vi "SpeedTokenizer.vi"(8 "error in (no error)":errorcluster, 11 "Command String":string) -> (0 "error out":errorcluster, 3 "Tokens":string[](array[string]))   [LabVIEW 2019, in "PathTokenizer.lvclass"]
uses:
  PathTokenizer.lvclass
  <vilib>/Utility/error.llb/whitespace.ctl
  <vilib>/regexp/Match Regular Expression.xnode
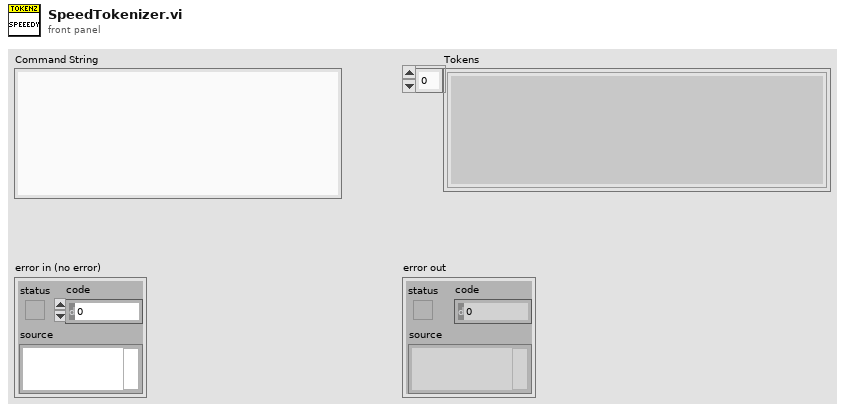
[diagram p1: front panel]
types:
  T1 = typedef "whitespace.ctl" = u16
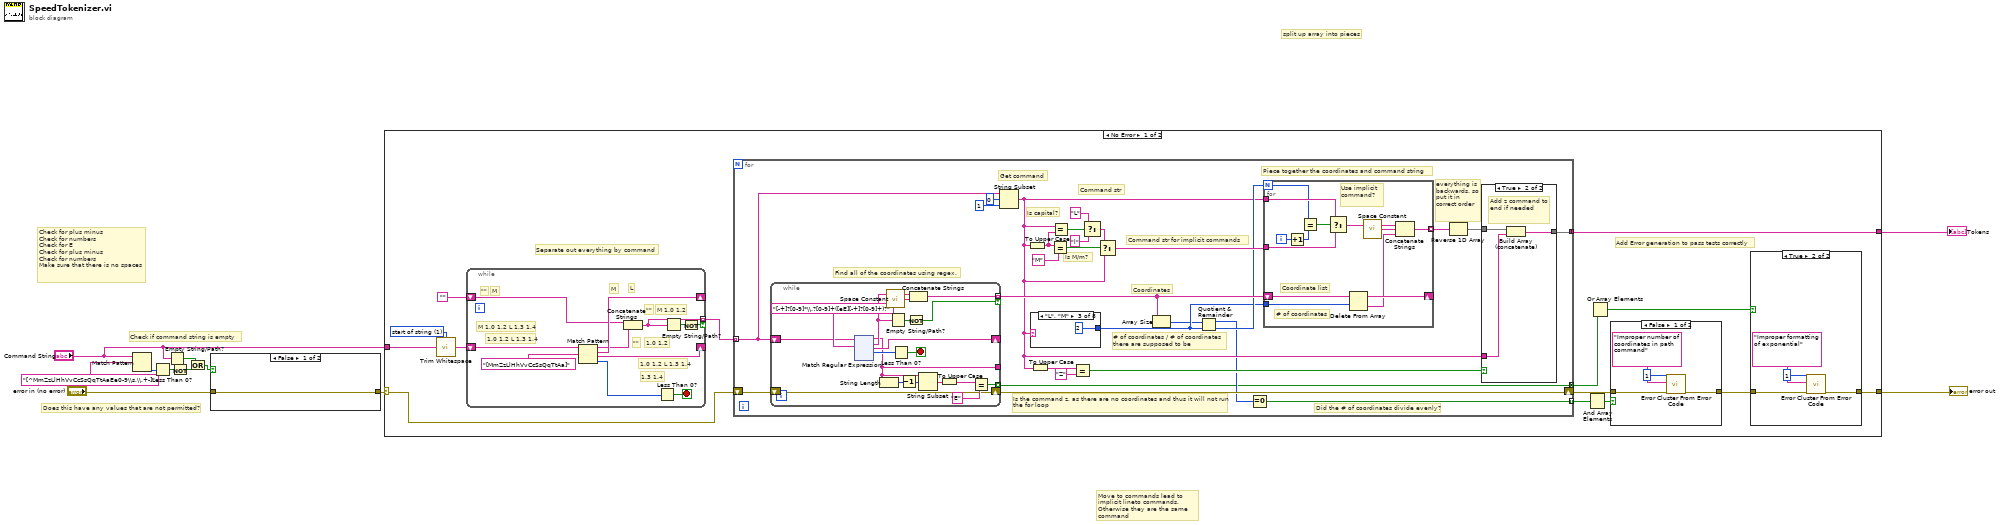
[diagram p0: block diagram]
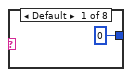
[diagram p5: hidden frame]
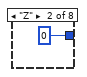
[diagram p6: hidden frame]
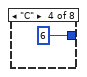
[diagram p7: hidden frame]
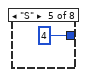
[diagram p8: hidden frame]
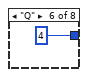
[diagram p9: hidden frame]
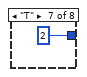
[diagram p10: hidden frame]
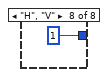
[diagram p11: hidden frame]
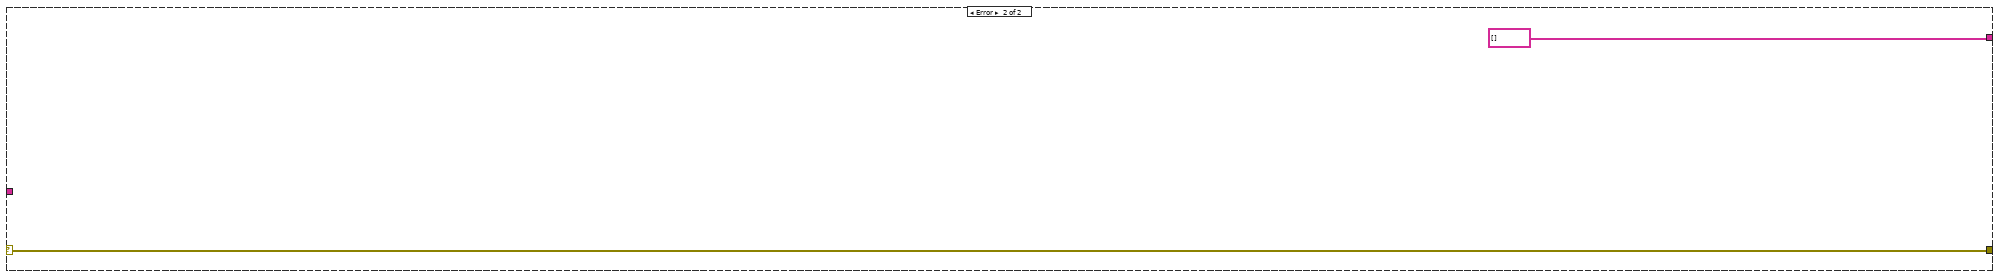
[diagram p12: hidden frame]
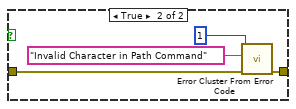
[diagram p13: hidden frame]
diagram:
  # "Check if command string is empty"
  # "Does this have any values that are not permitted?"
  # "Move to commands lead to implicit lineto commands. Otherwise they are the same command"
  # "split up array into pieces"
  # "Check for plus minus\nCheck for numbers\nCheck for E\nCheck for plus minus\nCheck for numbers\nMake sure that there is no spaces"
  n1 = Match Pattern(string="Command String", regular expression="[^MmZzLlHhVvCcSsQqTtAaEe0-9\\s,\\.+-]") -> (offset past match=w9:i32)  [unwired: 1 in, 3 out]
  n2 = Less Than 0?(x=w9) -> (x < 0?=w5:bool)
  n3 = Empty String/Path?(string/path="Command String") -> (empty?=w2:bool)
  n4 = Not(x=w5) -> (.not. x?=w4:bool)
  n5 = Or(x=w2, y=w4) -> (x .or. y?=w3:bool)
  n6 = case shown="False" w3 {
    tunnel: "error in (no error)" -> [w12 w14]
    tunnel: [w12 w13] -> w6
    frame False {
    }
    frame True {
      n7 = call <vilib>:"Error Cluster From Error Code.vi"("error in (no error)"=w14, "error message (\"\")"="Invalid Character in Path Command" ("error message (\"\")"), "error code (0)"=1) -> ("error out"=w13:errorcluster)  [unwired: 6 in]
    }
  }
  n8 = case shown="No Error" w6 {
    selector: w6 -> [w17 w236]
    tunnel: [w26 string[] []] -> w11
    tunnel: [w19 w236] -> w10
    tunnel: "Command String" -> [w25 _]
    frame No Error {
      w29 = T1 1 items=["both", "start of string", "end of string"] ("location (both)")
      # "Separate out everything by command"
      # "Add Error generation to pass tests correctly"
      n9 = call <vilib>:"Trim Whitespace.vi"("string"=w25, "location (both)"=w29) -> ("trimmed string"=w30:string)
      n10 = while {
        shift-right: [w225] -> _
        shift-left: w30 -> [w235]
        shift-right: [w233] -> _
        shift-left: "" -> [w232]
        tunnel: [w229] -> w28 mode=indexing if=w227
        stop <- w231 stop-if-true
        # "\"\""
        # "1.0 1.2 L 1.3 1.4"
        # "1.3 1.4"
        # "\"\""
        # "M 1.0 1.2"
        # "1.0 1.2"
        # "\"\""
        # "L"
        # "M"
        # "1.0 1.2 L 1.3 1.4"
        # "M"
        # "M 1.0 1.2 L 1.3 1.4"
        n11 = Match Pattern(string=w235, regular expression="[MmZzLlHhVvCcSsQqTtAa]") -> (before substring=w226:string, match substring=w233:string, after substring=w225:string, offset past match=w230:i32)  [unwired: 1 in]
        n12 = Concatenate Strings(w232, w226) -> (w229:string)
        n13 = Less Than 0?(x=w230) -> (x < 0?=w231:bool)
        n14 = Empty String/Path?(string/path=w229) -> (empty?=w228:bool)
        n15 = Not(x=w228) -> (.not. x?=w227:bool)
      }
      n16 = for {
        tunnel: w28 -> [w65] mode=indexing
        tunnel: [w51] -> w26 mode=concatenating
        shift-right: [w62] -> w22
        shift-left: w17 -> [w63]
        tunnel: [w42] -> w24 mode=indexing
        tunnel: [w41] -> w21 mode=concatenating
        # "everything is backwards, so put it in correct order"
        # "Piece together the coordinates and command string"
        # "Did the # of coordinates divide evenly?"
        # "Is the command z, as there are no coordinates and thus it will not run the for loop"
        # "Command str"
        # "Command str for implicit commands"
        # "Coordinates"
        # "# of coordinates / # of coordinates there are supposed to be"
        # "Get command"
        # "Find all of the coordinates using regex."
        # "Is M/m?"
        # "Is capital?"
        n17 = while {
          shift-right: [w108] -> _
          shift-left: w65 -> [w109]
          tunnel: [w102] -> w49 mode=indexing if=w101
          shift-right: [w94] -> w62
          shift-left: w63 -> [w94]
          tunnel: [w93] -> _
          tunnel: [w95] -> w41 mode=indexing
          stop <- w106 stop-if-true
          n18 = xnode "Match Regular Expression"("input string"=w109, "regular expression"="[-+]?[0-9]*\\.?[0-9]+([eE][-+]?[0-9]+)?") -> ("before match"=w93:string, "whole match"=w103:string, "after match"=w108:string, "offset past match"=w107:i32)  [unwired: 4 in, 1 out]
          n19 = String Length(string=w93) -> (length=w100:i32)
          n20 = call <vilib>:"Space Constant.vi"() -> ("String"=w104:string)
          n21 = Empty String/Path?(string/path=w103) -> (empty?=w105:bool)
          n22 = Less Than 0?(x=w107) -> (x < 0?=w106:bool)
          n23 = Decrement(x=w100) -> (x-1=w97:i32)
          n24 = Not(x=w105) -> (.not. x?=w101:bool)
          n25 = Concatenate Strings(w103, w104) -> (w102:string)
          n26 = String Subset(string=w93, offset (0)=w97) -> (substring=w99:string)  [unwired: 1 in]
          n27 = To Upper Case(1:w99) -> (0:w96:string)
          n28 = Equal?(x=w96, y="E") -> (x = y?=w95:bool)
        }
        n29 = String Subset(string=w65, offset (0)=0, length (rest)=1 ("length (rest)")) -> (substring=w45:string)
        n30 = To Upper Case(1:w45) -> (0:w59:string)
        n31 = case shown="\"L\", \"M\"" w45 {
          tunnel: [0 0 2 6 4 4 2 1] -> w46
          frame Default {
            # "There was an error handler here for unsupported command type"
          }
          frame "Z" {
          }
          frame "L", "M" {
          }
          frame "C" {
          }
          frame "S" {
          }
          frame "Q" {
          }
          frame "T" {
          }
          frame "H", "V" {
          }
        }
        n32 = To Upper Case(1:w45) -> (0:w54:string)
        n33 = Equal?(x=w59, y="M") -> (x = y?=w61:bool)
        n34 = Equal?(x=w45, y=w59) -> (x = y?=w58:bool)
        n35 = Equal?(x=w54, y="Z") -> (x = y?=w50:bool)
        n36 = Select(t="L", s=w58, f="l") -> (s? t:f=w55:string)
        n37 = Select(t=w55, s=w61, f=w45) -> (s? t:f=w48:string)
        n38 = Array Size(array=w49) -> (size(s)=w44:i32)
        n39 = Quotient & Remainder(x=w44, y=w46) -> (x-y*floor(x/y)=w43:i32, floor(x/y)=w47:i32)
        n40 = Equal To 0?(x=w43) -> (x = 0?=w42:bool)
        n41 = for {
          N: w47 -> [w72]
          tunnel: w46 -> [w82]
          shift-right: [w84] -> _
          shift-left: w49 -> [w83]
          tunnel: [w79] -> w64 mode=indexing
          tunnel: w45 -> [w76]
          tunnel: w48 -> [w78]
          i -> [w73]
          # "Use implicit command?"
          # "Coordinate list"
          # "# of coordinates"
          n42 = Increment(x=w73) -> (x+1=w74:i32)
          n43 = Equal?(x=w72, y=w74) -> (x = y?=w75:bool)
          n44 = Select(t=w76, s=w75, f=w78) -> (s? t:f=w77:string)
          n45 = Delete From Array(array=w83, length=w82) -> (deleted portion=w80:string[], array with subset deleted=w84:string[])  [unwired: 1 in]
          n46 = call <vilib>:"Space Constant.vi"() -> ("String"=w81:string)
          n47 = Concatenate Strings(w77, w81, w80) -> (w79:string)
        }
        n48 = Reverse 1D Array(array=w64) -> (reversed array=w52:string[])
        n49 = case shown="True" w50 {
          tunnel: w52 -> [w68 w70]
          tunnel: [w68 w69] -> w51
          tunnel: w45 -> [_ w71]
          frame False {
          }
          frame True {
            # "Add z command to end if needed"
            n50 = Build Array (concatenate)(w70, w71) -> (w69:string[])
          }
        }
      }
      n51 = And Array Elements(Boolean array=w24) -> (logical AND=w23:bool)
      n52 = Or Array Elements(Boolean array=w21) -> (logical OR=w18:bool)
      n53 = case shown="False" w23 {
        tunnel: w22 -> [w39 w40]
        tunnel: [w38 w40] -> w20
        frame False {
          n54 = call <vilib>:"Error Cluster From Error Code.vi"("error in (no error)"=w39, "error message (\"\")"="Improper number of coordinates in path command" ("error message (\"\")"), "error code (0)"=1) -> ("error out"=w38:errorcluster)  [unwired: 6 in]
        }
        frame True {
        }
      }
      n55 = case shown="True" w18 {
        tunnel: w20 -> [w31 w35]
        tunnel: [w31 w34] -> w19
        frame False {
        }
        frame True {
          n56 = call <vilib>:"Error Cluster From Error Code.vi"("error in (no error)"=w35, "error message (\"\")"="Improper formatting of exponential" ("error message (\"\")"), "error code (0)"=1) -> ("error out"=w34:errorcluster)  [unwired: 6 in]
        }
      }
    }
    frame Error {
    }
  }
  "error out" <- w10
  "Tokens" <- w11
